vi "Handle Error.vi"(8 "error in":errorcluster, 11 "Runner in":refnum<class "Runner.lvclass">) -> (0 "error out":errorcluster, 2 "stop actor?":bool=TRUE, 3 "Runner out":refnum<class "Runner.lvclass">)   [LabVIEW 2026, in "Runner.lvlib" / "Runner.lvclass"]
doc: "<p>(<strong>Filename</strong>: <span class=\"dnl\">Actor Framework.lvlib:Actor.lvclass:Handle Error.vi</span>)</p>\n<p>Defines how the actor handles an error that occurred while processing a message. By default, this method does nothing except stop the actor.</p>"
uses:
  Runner.lvclass
  Runner.lvclass/Runner.ctl
  <vilib>/ActorFramework/Actor/Actor.lvclass
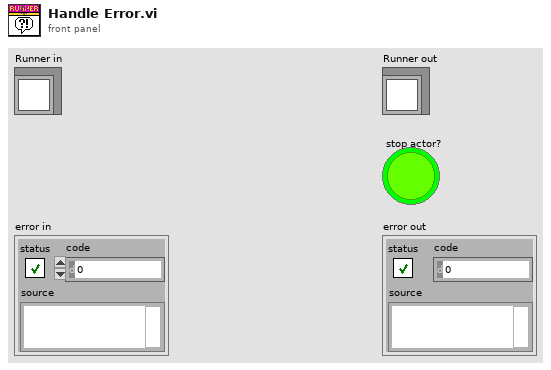
[diagram p1: front panel]
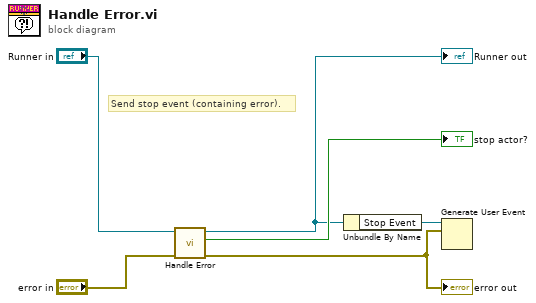
[diagram p0: block diagram]
diagram:
  # "Send stop event (containing error)."
  n1 = call-parent "Handle Error.vi"("error in (no error)"="error in", "Actor in"="Runner in") -> ("error out"=w5:errorcluster, "stop actor?"=→"stop actor?":bool, "Actor out"=w2:refnum<class "Runner.lvclass">)  [unwired: 7 in]
  "Runner out" <- w2
  "error out" <- w5
  n2 = Unbundle By Name(w2) -> ("Stop Event"=w1:refnum<user-event>)
  n3 = Generate User Event(user event=w1, event data cluster=w5) -> ()  [unwired: 2 in, 2 out]
